vi "2636 EPSC fixed log time version.vi"() -> ()   [LabVIEW 2023]
uses:
  <instrlib>/Keithley 2600 Series/Public/Channel.ctl
  <instrlib>/Keithley 2600 Series/Keithley 2600 Series.lvlib
  <userlib>/_OpenG.lib/time/time.llb/openg_time.lvlib
panel:
  in  "Down Sample Factor":u8=3
  out "EPSC":cluster{"X":dbl[], "Y":dbl[]}[](graph)
  out "Log Time (s)":dbl=5000.0
  out "Gate Pulse":cluster{"X":dbl[], "Y":dbl[]}[](graph)
  in  "error in (no error)":errorcluster
  in  "Log Time Before Pulse (s)":dbl=0.5 format="%#_13g"
  in  "Log Time After Pulses (s)":dbl=10.0 format="%#_13g"
  in  "Auto Enable Output":bool=TRUE
  in  "Reset":bool=TRUE
  in  "Error Query":bool
  out "I_ds Points":i32=5000
  out "Pulsed IV Filename Out":path caption="Filename Out"
  in  "Pulsed IV Filename":path=path "C:/Data/pulse_I_V.lvm" caption="Filename"
  out "Pulse IV":cluster{"X":dbl[], "Y":dbl[]}[](graph)
  out "I_ds Log Filename Out":path caption="Filename Out"
  in  "I_ds Log Filename":path=path "C:/Data/I_ds_vs_time.lvm" caption="Filename"
  out "Data":dbl[](array[numeric])
  out "error out":errorcluster
  out "Complete?":bool
  out "Overrun?":bool
  out "Overflow?":bool
  in  "Stop":bool
  in  "Pulse Duration (s)":dbl=0.01
  in  "Post-Pulse Duration (s)":dbl=0.05
  in  "Pre-Pulse Duration (s)":dbl=0.05
  in  "Buffer size":u32=1024
  in  "Pulse Number":u32=10
  in  "Drain Source Channel":T1=enum."Channel B"
  in  "V_ds(V)":dbl=0.01
  in  "I_ds NPLC":dbl=0.1
  in  "I_ds Range (A)":dbl=1e-06
  in  "I pulse Range (A)":dbl=1e-06
  in  "I pulse NPLC":dbl=0.1
  in  "Pulse Level (V)":dbl=15.0
  in  "Pulse Channel":T1
  in  "2636 Address":refnum<visa-resource-name>="GPIB0::26::INSTR"
  # "Synaptic EPSC Measurement (Three-terminal Devices)"
  # "by JHC (20250308)"
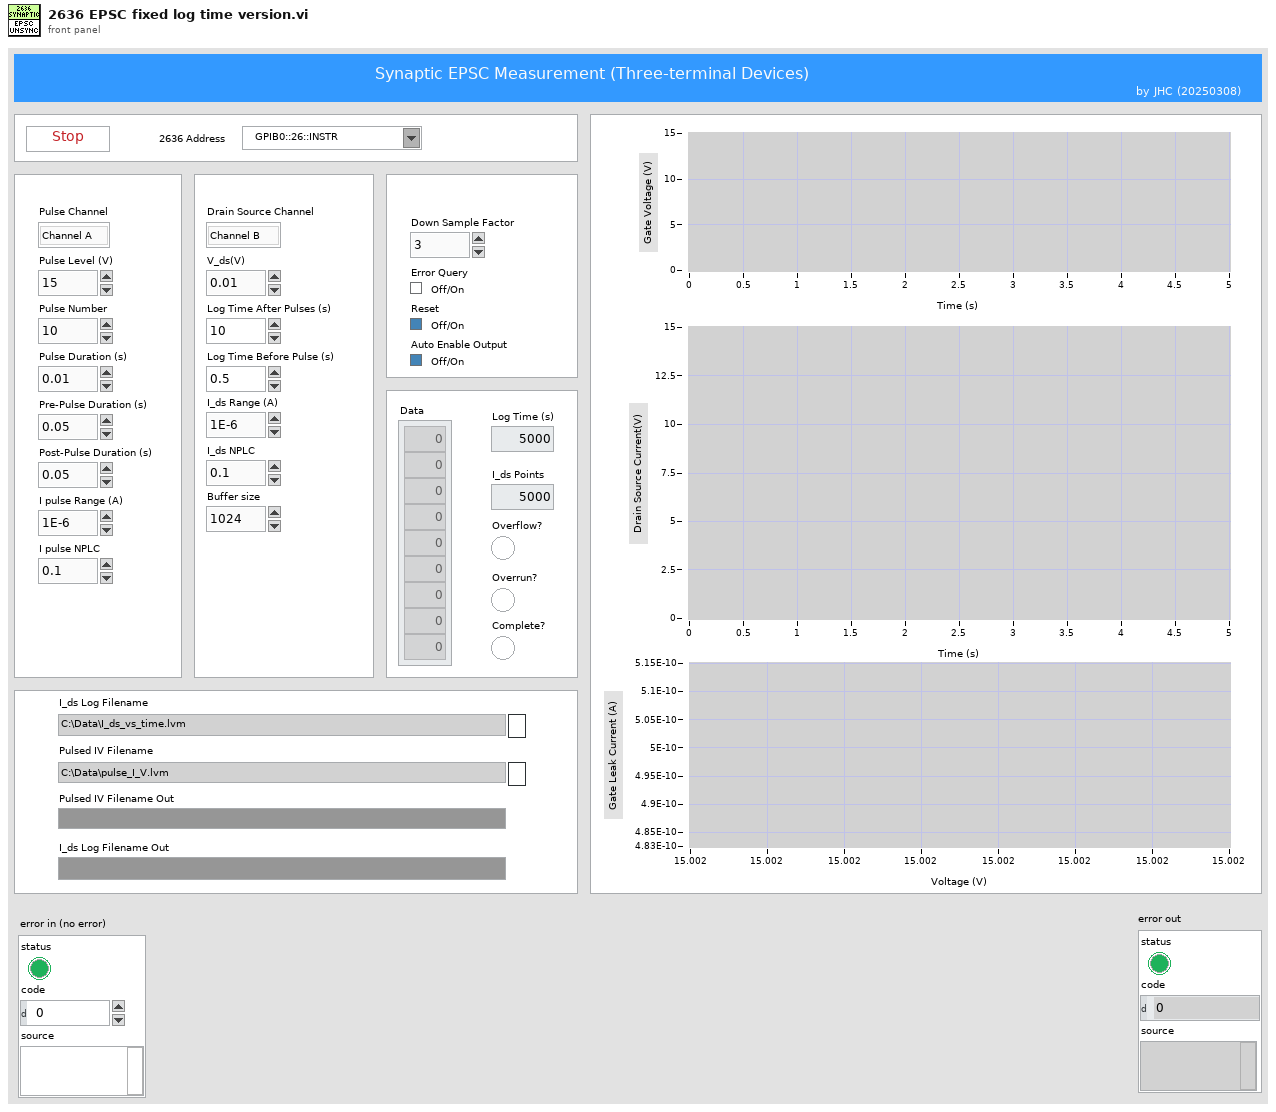
[diagram p1: front panel]
types:
  T1 = typedef "Keithley 2600 Series.lvlib/Channel.ctl" = enum32{"Channel A", "Channel B"}
  T2 = enum16{"None/Disconnect", "Digital I/O Trigger", "TSP-Link Trigger", "LAN Trigger", "Blender", "Timer Expired", "Front Panel Trigger", "Software Trigger", "SMU Sweeping", "SMU Armed", "SMU Source Complete", "SMU Measure Complete", "SMU Pulse Complete", "SMU Sweep Complete", "SMU Idle"}
  T3 = enum16{"Current", "Voltage", "IV", "Resistance", "Power"}
  T4 = enum32{"ASCII", "Real 32", "Real 64", "Single Precision Real", "Double Precision Real"}
  T5 = enum16{"Digital I/O", "TSP-Link", "LAN", "Blender", "Timer", "Arm", "Source", "Measure", "End Pulse"}
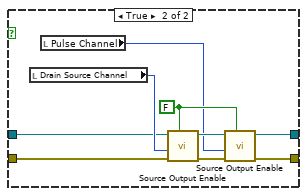
[diagram p2: hidden frame]
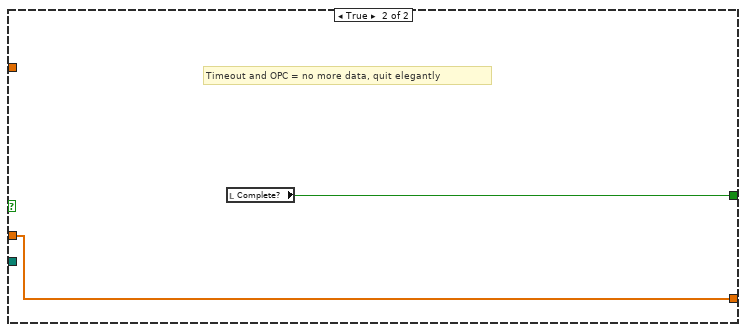
[diagram p5: hidden frame]
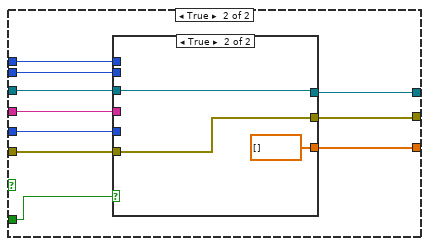
[diagram p8: hidden frame]
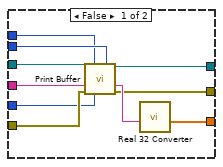
[diagram p9: hidden frame]
diagram:
  w25 = 0.0 ("element")
  w41 = sgl[] [] ("Data Array Out")
  w44 = u16 1 items=["Channel A", "Channel B"] ("Channel (Channel A)")
  w45 = u16 0 items=["Channel A", "Channel B"] ("Channel (Channel A)")
  w62 = u16 0 items=["Current", "Voltage", "Resistance", "Power"] ("Function (Current)")
  w70 = u16 2 items=["Channel A", "Channel B", "Channels A & B", "User"] ("Screen (Channels A & B)")
  # "Wait 1s"
  # "Start Pulse SMU"
  # "Start DS SMU"
  n1 = call <instrlib>:"Initialize.vi"("Reset (True)"="Reset", "error in (no error)"="error in (no error)", "Error Query (False)"="Error Query", "ID Query (True)"=TRUE, "VISA resource name"="2636 Address") -> ("error out"=w27:errorcluster, "VISA resource name out"=w30:refnum<visa-resource-name>)  [unwired: 5 in]
  n2 = call <instrlib>:"Error Queue Clear.vi"("error in (no error)"=w27, "VISA resource name"=w30) -> ("error out"=w28:errorcluster, "VISA resource name out"=w29:refnum<visa-resource-name>)  [unwired: 6 in, 2 out]
  n3 = call <instrlib>:"Abort SMU Op.vi"("error in"=w28, "Channel (Channel A)"=w45, "VISA resource name"=w29) -> ("error out"=w46:errorcluster, "VISA resource name out"=w47:refnum<visa-resource-name>)  [unwired: 5 in, 2 out]
  n4 = call <instrlib>:"Abort SMU Op.vi"("error in"=w46, "Channel (Channel A)"=w44, "VISA resource name"=w47) -> ("error out"=w42:errorcluster, "VISA resource name out"=w43:refnum<visa-resource-name>)  [unwired: 5 in, 2 out]
  n5 = call <instrlib>:"Reset SMU.vi"("SMU B (No)"="Reset", "SMU A (No)"="Reset", "error in (no error)"=w42, "VISA resource name"=w43) -> ("error out"=w109:errorcluster, "VISA resource name out"=w110:refnum<visa-resource-name>)  [unwired: 4 in, 2 out]
  n6 = flat-sequence {
    tunnel: w110 -> [w143]
    tunnel: w109 -> [w142]
    tunnel: [w124] -> w108
    tunnel: [w123] -> w107
    tunnel: w108 -> [w182]
    tunnel: w107 -> [w183]
    tunnel: [w181] -> w106
    tunnel: [w180] -> w105
    tunnel: w106 -> [w223]
    tunnel: w105 -> [w221]
    tunnel: [w202] -> w104
    tunnel: [w201] -> w103
    tunnel: w104 -> [w301]
    tunnel: w103 -> [w300]
    tunnel: [w268] -> w102
    tunnel: [w267] -> w101
    tunnel: [w253] -> w100
    tunnel: w102 -> [w326]
    tunnel: w101 -> [w327]
    tunnel: w100 -> [w352]
    tunnel: [w330] -> w99
    tunnel: [w329] -> w98
    tunnel: w99 -> [w360]
    tunnel: w98 -> [w359]
    tunnel: [w356] -> w67
    tunnel: [w355] -> w66
    frame #0 {
      w131 = enum32{"Current", "Voltage"}."Current" ("Function (Current)")
      w132 = FALSE ("Autorange (On)")
      w112 = enum32{"Current", "Voltage"}."Voltage" ("Function (Current)")
      # "Init Pulse Gate Channel"
      n7 = call <instrlib>:"Source Function.vi"("Function (Current)"=w112, "error in (no error)"=w142, "Channel (Channel A)"="Pulse Channel", "VISA resource name"=w143) -> ("error out"=w144:errorcluster, "VISA resource name out"=w145:refnum<visa-resource-name>)  [unwired: 4 in, 2 out]
      n8 = call <instrlib>:"Source Level.vi"("Level (0.000)"=0.0, "Function (Current)"=w112, "error in (no error)"=w144, "Channel (Channel A)"="Pulse Channel", "VISA resource name"=w145) -> ("error out"=w140:errorcluster, "VISA resource name out"=w141:refnum<visa-resource-name>)  [unwired: 3 in, 2 out]
      n9 = call <instrlib>:"Source Autorange.vi"("Autorange (On)"=w132, "Function (Current)"=w112, "error in (no error)"=w140, "Channel (Channel A)"="Pulse Channel", "VISA resource name"=w141) -> ("error out"=w138:errorcluster, "VISA resource name out"=w139:refnum<visa-resource-name>)  [unwired: 3 in, 2 out]
      n10 = local read "Pulse Level (V)"() -> (w111:dbl)
      n11 = call <instrlib>:"Source Autorange.vi"("Autorange (On)"=w132, "Function (Current)"=w131, "error in (no error)"=w138, "Channel (Channel A)"="Pulse Channel", "VISA resource name"=w139) -> ("error out"=w119:errorcluster, "VISA resource name out"=w121:refnum<visa-resource-name>)  [unwired: 3 in, 2 out]
      n12 = call <instrlib>:"Source Range.vi"("Range (1.000)"=w111, "Function (Current)"=w112, "error in (no error)"=w119, "Channel (Channel A)"="Pulse Channel", "VISA resource name"=w121) -> ("error out"=w118:errorcluster, "VISA resource name out"=w120:refnum<visa-resource-name>)  [unwired: 3 in, 2 out]
      n13 = call <instrlib>:"Measure NPLC.vi"("NPLC (1.000)"="I pulse NPLC", "error in (no error)"=w118, "Channel (Channel A)"="Pulse Channel", "VISA resource name"=w120) -> ("error out"=w136:errorcluster, "VISA resource name out"=w133:refnum<visa-resource-name>)  [unwired: 4 in, 2 out]
      n14 = call <instrlib>:"Measure Autorange.vi"("Autorange (On)"=w132, "Function (Current)"=w112, "error in (no error)"=w136, "Channel (Channel A)"="Pulse Channel", "VISA resource name"=w133) -> ("error out"=w135:errorcluster, "VISA resource name out"=w134:refnum<visa-resource-name>)  [unwired: 3 in, 2 out]
      n15 = call <instrlib>:"Measure Autorange.vi"("Autorange (On)"=w132, "Function (Current)"=w131, "error in (no error)"=w135, "Channel (Channel A)"="Pulse Channel", "VISA resource name"=w134) -> ("error out"=w117:errorcluster, "VISA resource name out"=w116:refnum<visa-resource-name>)  [unwired: 3 in, 2 out]
      n16 = call <instrlib>:"Measure Range.vi"("Range (1.000)"=w111, "Function (Current)"=w112, "error in (no error)"=w117, "Channel (Channel A)"="Pulse Channel", "VISA resource name"=w116) -> ("error out"=w114:errorcluster, "VISA resource name out"=w115:refnum<visa-resource-name>)  [unwired: 3 in, 2 out]
      n17 = call <instrlib>:"Measure Range.vi"("Range (1.000)"="I pulse Range (A)", "Function (Current)"=w131, "error in (no error)"=w114, "Channel (Channel A)"="Pulse Channel", "VISA resource name"=w115) -> ("error out"=w129:errorcluster, "VISA resource name out"=w128:refnum<visa-resource-name>)  [unwired: 3 in, 2 out]
      n18 = call <instrlib>:"Measure Sense Mode.vi"("error in (no error)"=w129, "Channel (Channel A)"="Pulse Channel", "VISA resource name"=w128) -> ("error out"=w126:errorcluster, "VISA resource name out"=w127:refnum<visa-resource-name>)  [unwired: 2 in, 5 out]
      n19 = call <instrlib>:"Measure Autozero.vi"("Autozero (Auto)"=enum32{"Off", "Once", "Auto"}."Once", "error in (no error)"=w126, "Channel (Channel A)"="Pulse Channel", "VISA resource name"=w127) -> ("error out"=w123:errorcluster, "VISA resource name out"=w124:refnum<visa-resource-name>)  [unwired: 1 in, 5 out]
    }
    frame #1 {
      w165 = 0.0 ("Interval (0.000)")
      w185 = enum32{"Current", "Voltage"}."Current" ("Function (Current)")
      w184 = FALSE ("Autorange (On)")
      w171 = enum32{"Current", "Voltage"}."Voltage" ("Function (Current)")
      # "50HZ"
      # "Init Drain Source Channel"
      n20 = local read "Log Time After Pulses (s)"() -> (w153:dbl)
      n21 = local read "Log Time Before Pulse (s)"() -> (w147:dbl)
      n22 = local read "Pulse Number"() -> (w152:u32)
      n23 = local read "Pre-Pulse Duration (s)"() -> (w148:dbl)
      n24 = local read "Pulse Duration (s)"() -> (w149:dbl)
      n25 = local read "Post-Pulse Duration (s)"() -> (w150:dbl)
      n26 = Compound Arithmetic op=ADD(w148, w149, w150) -> (w151:dbl)
      n27 = call <instrlib>:"Source Function.vi"("Function (Current)"=w171, "error in (no error)"=w183, "Channel (Channel A)"="Drain Source Channel", "VISA resource name"=w182) -> ("error out"=w199:errorcluster, "VISA resource name out"=w200:refnum<visa-resource-name>)  [unwired: 4 in, 2 out]
      n28 = Multiply(x=w152, y=w151) -> (x*y=w154:dbl)
      n29 = call <instrlib>:"Source Level.vi"("Level (0.000)"="V_ds(V)", "Function (Current)"=w171, "error in (no error)"=w199, "Channel (Channel A)"="Drain Source Channel", "VISA resource name"=w200) -> ("error out"=w197:errorcluster, "VISA resource name out"=w198:refnum<visa-resource-name>)  [unwired: 3 in, 2 out]
      n30 = Compound Arithmetic op=ADD(w153, w147, w154) -> (w146:dbl)
      "Log Time (s)" <- w146
      n31 = call <instrlib>:"Source Autorange.vi"("Autorange (On)"=w184, "Function (Current)"=w171, "error in (no error)"=w197, "Channel (Channel A)"="Drain Source Channel", "VISA resource name"=w198) -> ("error out"=w195:errorcluster, "VISA resource name out"=w196:refnum<visa-resource-name>)  [unwired: 3 in, 2 out]
      n32 = local read "I_ds NPLC"() -> (w159:dbl)
      n33 = call <instrlib>:"Source Autorange.vi"("Autorange (On)"=w184, "Function (Current)"=w185, "error in (no error)"=w195, "Channel (Channel A)"="Drain Source Channel", "VISA resource name"=w196) -> ("error out"=w179:errorcluster, "VISA resource name out"=w176:refnum<visa-resource-name>)  [unwired: 3 in, 2 out]
      n34 = Multiply(x=0.02, y=w159) -> (x*y=w157:dbl)
      n35 = call <instrlib>:"Source Range.vi"("Range (1.000)"="V_ds(V)", "Function (Current)"=w171, "error in (no error)"=w179, "Channel (Channel A)"="Drain Source Channel", "VISA resource name"=w176) -> ("error out"=w178:errorcluster, "VISA resource name out"=w177:refnum<visa-resource-name>)  [unwired: 3 in, 2 out]
      n36 = Divide(x=w146, y=w157) -> (x/y=w156:dbl)
      n37 = call <instrlib>:"Measure NPLC.vi"("NPLC (1.000)"="I_ds NPLC", "error in (no error)"=w178, "Channel (Channel A)"="Drain Source Channel", "VISA resource name"=w177) -> ("error out"=w166:errorcluster, "VISA resource name out"=w167:refnum<visa-resource-name>)  [unwired: 4 in, 2 out]
      n38 = To Long Integer(number=w156) -> (32bit integer=w155:i32)
      "I_ds Points" <- w155
      n39 = call <instrlib>:"Measure Interval.vi"("Interval (0.000)"=w165, "error in (no error)"=w166, "Channel (Channel A)"="Drain Source Channel", "VISA resource name"=w167) -> ("error out"=w169:errorcluster, "VISA resource name out"=w168:refnum<visa-resource-name>)  [unwired: 4 in, 2 out]
      n40 = call <instrlib>:"Measure Delay.vi"("Delay (0)"=w165, "error in (no error)"=w169, "Channel (Channel A)"="Drain Source Channel", "VISA resource name"=w168) -> ("error out"=w163:errorcluster, "VISA resource name out"=w164:refnum<visa-resource-name>)  [unwired: 4 in, 2 out]
      n41 = call <instrlib>:"Measure Count.vi"("Count (1)"=w155, "error in (no error)"=w163, "Channel (Channel A)"="Drain Source Channel", "VISA resource name"=w164) -> ("error out"=w161:errorcluster, "VISA resource name out"=w162:refnum<visa-resource-name>)  [unwired: 4 in, 2 out]
      n42 = call <instrlib>:"Measure Autorange.vi"("Autorange (On)"=w184, "Function (Current)"=w171, "error in (no error)"=w161, "Channel (Channel A)"="Drain Source Channel", "VISA resource name"=w162) -> ("error out"=w193:errorcluster, "VISA resource name out"=w192:refnum<visa-resource-name>)  [unwired: 3 in, 2 out]
      n43 = call <instrlib>:"Measure Autorange.vi"("Autorange (On)"=w184, "Function (Current)"=w185, "error in (no error)"=w193, "Channel (Channel A)"="Drain Source Channel", "VISA resource name"=w192) -> ("error out"=w172:errorcluster, "VISA resource name out"=w173:refnum<visa-resource-name>)  [unwired: 3 in, 2 out]
      n44 = call <instrlib>:"Measure Range.vi"("Range (1.000)"="V_ds(V)", "Function (Current)"=w171, "error in (no error)"=w172, "Channel (Channel A)"="Drain Source Channel", "VISA resource name"=w173) -> ("error out"=w175:errorcluster, "VISA resource name out"=w174:refnum<visa-resource-name>)  [unwired: 3 in, 2 out]
      n45 = call <instrlib>:"Measure Range.vi"("Range (1.000)"="I_ds Range (A)", "Function (Current)"=w185, "error in (no error)"=w175, "VISA resource name"=w174) -> ("error out"=w190:errorcluster, "VISA resource name out"=w189:refnum<visa-resource-name>)  [unwired: 4 in, 2 out]
      n46 = call <instrlib>:"Measure Sense Mode.vi"("error in (no error)"=w190, "Channel (Channel A)"="Drain Source Channel", "VISA resource name"=w189) -> ("error out"=w187:errorcluster, "VISA resource name out"=w188:refnum<visa-resource-name>)  [unwired: 2 in, 5 out]
      n47 = call <instrlib>:"Measure Autozero.vi"("Autozero (Auto)"=enum32{"Off", "Once", "Auto"}."Once", "error in (no error)"=w187, "Channel (Channel A)"="Drain Source Channel", "VISA resource name"=w188) -> ("error out"=w181:errorcluster, "VISA resource name out"=w180:refnum<visa-resource-name>)  [unwired: 1 in, 5 out]
    }
    frame #2 {
      w215 = TRUE ("Append Mode (Off)")
      w214 = "v_ds" ("Buffer Name (buf)")
      w216 = TRUE ("Append Mode (Off)")
      w218 = "i_ds" ("Buffer Name (buf)")
      w227 = FALSE ("Collect Timestamps (Off)")
      w226 = "pulse_iv_table.v" ("Buffer Name (buf)")
      w225 = TRUE ("Append Mode (Off)")
      w224 = "pulse_iv_table.i" ("Buffer Name (buf)")
      # "set up circular buffer"
      # "A large size"
      # "Init Buffer"
      n48 = local read "Pulse Channel"() -> (w242:T1)
      n49 = VISA Write(VISA resource name=w221, write buffer="pulse_iv_table = {}\nds_iv_table = {}", error in (no error)=w223) -> (VISA resource name out=w228:refnum<visa-resource-name>, error out=w229:errorcluster)  [unwired: 1 out]
      n50 = call <instrlib>:"Error Query.vi"("error in (no error)"=w229, "VISA resource name"=w228) -> ("error out"=w241:errorcluster, "VISA resource name out"=w240:refnum<visa-resource-name>)  [unwired: 8 out]
      n51 = call <instrlib>:"Buffer Make Buffer.vi"("Capacity (1)"="Pulse Number", "Channel (Channel A)"=w242, "error in (no error)"=w241, "Buffer Name (buf)"=w224, "VISA resource name"=w240) -> ("error out"=w230:errorcluster, "VISA resource name out"=w231:refnum<visa-resource-name>)  [unwired: 1 in, 4 out]
      n52 = call <instrlib>:"Buffer Clear.vi"("error in (no error)"=w230, "Buffer Name"=w224, "VISA resource name"=w231) -> ("error out"=w233:errorcluster, "VISA resource name out"=w232:refnum<visa-resource-name>)  [unwired: 7 out]
      n53 = call <instrlib>:"Buffer Configure.vi"("Collect Timestamps (Off)"=w227, "error in (no error)"=w233, "Buffer Name"=w224, "Append Mode (Off)"=w225, "VISA resource name"=w232) -> ("error out"=w235:errorcluster, "VISA resource name out"=w234:refnum<visa-resource-name>)  [unwired: 2 in, 3 out]
      n54 = call <instrlib>:"Buffer Make Buffer.vi"("Capacity (1)"="Pulse Number", "Channel (Channel A)"=w242, "error in (no error)"=w235, "Buffer Name (buf)"=w226, "VISA resource name"=w234) -> ("error out"=w237:errorcluster, "VISA resource name out"=w236:refnum<visa-resource-name>)  [unwired: 1 in, 4 out]
      n55 = call <instrlib>:"Buffer Clear.vi"("error in (no error)"=w237, "Buffer Name"=w226, "VISA resource name"=w236) -> ("error out"=w239:errorcluster, "VISA resource name out"=w238:refnum<visa-resource-name>)  [unwired: 7 out]
      n56 = call <instrlib>:"Buffer Configure.vi"("Collect Source Values (Off)"=w227, "error in (no error)"=w239, "Buffer Name"=w226, "Append Mode (Off)"=w225, "VISA resource name"=w238) -> ("error out"=w249:errorcluster, "VISA resource name out"=w248:refnum<visa-resource-name>)  [unwired: 2 in, 3 out]
      n57 = local read "Drain Source Channel"() -> (w206:T1)
      n58 = call <instrlib>:"Buffer Make Buffer.vi"("Capacity (1)"="Buffer size", "Channel (Channel A)"=w206, "error in (no error)"=w249, "Buffer Name (buf)"=w218, "VISA resource name"=w248) -> ("error out"=w245:errorcluster, "VISA resource name out"=w244:refnum<visa-resource-name>)  [unwired: 1 in, 4 out]
      n59 = call <instrlib>:"Buffer Clear.vi"("error in (no error)"=w245, "Buffer Name"=w218, "VISA resource name"=w244) -> ("error out"=w247:errorcluster, "VISA resource name out"=w246:refnum<visa-resource-name>)  [unwired: 7 out]
      n60 = call <instrlib>:"Buffer Configure.vi"("Collect Timestamps (Off)"=w216, "error in (no error)"=w247, "Buffer Name"=w218, "Append Mode (Off)"=w216, "VISA resource name"=w246) -> ("error out"=w220:errorcluster, "VISA resource name out"=w219:refnum<visa-resource-name>)  [unwired: 2 in, 3 out]
      n61 = call <instrlib>:"Advanced Buffer Configuration.vi"("VISA resource name"=w219, "Enable Buffer Cache Mode (Disable)"=w216, "Buffer Name"=w218, "Buffer Fill Mode (Fill_Once)"=enum16{"FILL_ONCE", "FILL_WINDOW"}."FILL_WINDOW", "error in (no error)"=w220) -> ("VISA resource name out"=w204:refnum<visa-resource-name>, "error out"=w203:errorcluster)  [unwired: 9 in]
      n62 = call <instrlib>:"Buffer Make Buffer.vi"("Capacity (1)"="Buffer size", "Channel (Channel A)"=w206, "error in (no error)"=w203, "Buffer Name (buf)"=w214, "VISA resource name"=w204) -> ("error out"=w210:errorcluster, "VISA resource name out"=w211:refnum<visa-resource-name>)  [unwired: 1 in, 4 out]
      n63 = call <instrlib>:"Buffer Clear.vi"("error in (no error)"=w210, "Buffer Name"=w214, "VISA resource name"=w211) -> ("error out"=w208:errorcluster, "VISA resource name out"=w209:refnum<visa-resource-name>)  [unwired: 7 out]
      n64 = call <instrlib>:"Buffer Configure.vi"("Collect Timestamps (Off)"=w215, "error in (no error)"=w208, "Buffer Name"=w214, "Append Mode (Off)"=w215, "VISA resource name"=w209) -> ("error out"=w212:errorcluster, "VISA resource name out"=w213:refnum<visa-resource-name>)  [unwired: 2 in, 3 out]
      n65 = call <instrlib>:"Advanced Buffer Configuration.vi"("VISA resource name"=w213, "Enable Buffer Cache Mode (Disable)"=w215, "Buffer Name"=w214, "Buffer Fill Mode (Fill_Once)"=enum16{"FILL_ONCE", "FILL_WINDOW"}."FILL_WINDOW", "error in (no error)"=w212) -> ("VISA resource name out"=w201:refnum<visa-resource-name>, "error out"=w202:errorcluster)  [unwired: 9 in]
    }
    frame #3 {
      w257 = u32 4 ("Timer Number (1)")
      w271 = u32 1 ("Timer Number (1)")
      w283 = u32 3 ("Timer Number (1)")
      w307 = u32 2 ("Timer Number (1)")
      # "SMU Armed when timer4 expires"
      # "Trigger timer4 when the SMU Sweeping, only once"
      # "Trigger timer1 when the SMU Armed, repeat N times"
      # "Trigger end pulse after timer3 expired"
      # "Configure measure action (default is 0) to start after source immediately"
      # "set source pulse level and end pusle idle"
      # "Trigger timer3 when the SMU source pulse level"
      # "Create a fixed level voltage sweep"
      # "Configure source action to start after timer2 expired"
      # "Trigger timer2 when timer1 expired or first run."
      # "Init Trigger Model (Pulse Channel)"
      n66 = local read "Pulse Channel"() -> (w253:T1)
      n67 = Pick Line(multi-line string="smua\nsmub", line index=w253) -> (output string=w266:string)  [unwired: 1 in]
      n68 = Format Into String(format string="%s.trigger.source.listv({%f})\\n", w266, "Pulse Level (V)") -> (resulting string=w304:string)  [unwired: 2 in, 1 out]
      n69 = call <instrlib>:"Format Event ID.vi"("Channel (Channel A)"=w253, "Event Type (None)"=T2."SMU Sweeping") -> ("Event ID"=w261:string)  [unwired: 8 in, 1 out]
      n70 = Format Into String(format string="%s.trigger.source.action = %s.ENABLE\n%s.trigger.endpulse.action = %s.SOURCE_IDLE", initial string=w304, w266, w266, w266, w266) -> (resulting string=w299:string)  [unwired: 1 in, 1 out]
      n71 = VISA Write(VISA resource name=w300, write buffer=w299, error in (no error)=w301) -> (VISA resource name out=w263:refnum<visa-resource-name>, error out=w262:errorcluster)  [unwired: 1 out]
      n72 = call <instrlib>:"Config Timer.vi"("VISA resource name"=w263, "Delay (1e-3)"="Log Time Before Pulse (s)", "Timer Number (1)"=w257, "error in"=w262, "Input Event"=w261) -> ("VISA resource name out"=w259:refnum<visa-resource-name>, "error out"=w255:errorcluster)  [unwired: 7 in, 2 out]
      n73 = call <instrlib>:"Format Event ID.vi"("Event Module # (1)"=w257, "Event Type (None)"=T2."Timer Expired") -> ("Event ID"=w256:string)  [unwired: 8 in, 1 out]
      n74 = call <instrlib>:"Config Arm Event.vi"("Arm Input Event"=w256, "error in"=w255, "Channel (Channel A)"=w253, "VISA resource name"=w259) -> ("error out"=w251:errorcluster, "VISA resource name out"=w250:refnum<visa-resource-name>)  [unwired: 4 in, 2 out]
      n75 = call <instrlib>:"Format Event ID.vi"("Channel (Channel A)"=w253, "Event Type (None)"=T2."SMU Armed") -> ("Event ID"=w252:string)  [unwired: 8 in, 1 out]
      n76 = local read "Pre-Pulse Duration (s)"() -> (w280:dbl)
      n77 = local read "Pulse Number"() -> (w276:u32)
      n78 = local read "Pulse Duration (s)"() -> (w281:dbl)
      n79 = Decrement(x=w276) -> (x-1=w272:u32)
      n80 = Compound Arithmetic op=ADD(w281, w280, "Post-Pulse Duration (s)") -> (w278:dbl)
      n81 = call <instrlib>:"Config Timer.vi"("VISA resource name"=w250, "Count (1)"=w272, "Delay (1e-3)"=w278, "Timer Number (1)"=w271, "Passthrough (Off)"=TRUE, "error in"=w251, "Input Event"=w252) -> ("VISA resource name out"=w273:refnum<visa-resource-name>, "error out"=w274:errorcluster)  [unwired: 5 in, 2 out]
      n82 = call <instrlib>:"Format Event ID.vi"("Event Module # (1)"=w271, "Event Type (None)"=T2."Timer Expired") -> ("Event ID"=w311:string)  [unwired: 8 in, 1 out]
      n83 = call <instrlib>:"Config Timer.vi"("VISA resource name"=w273, "Delay (1e-3)"="Pre-Pulse Duration (s)", "Timer Number (1)"=w307, "error in"=w274, "Input Event"=w311) -> ("VISA resource name out"=w310:refnum<visa-resource-name>, "error out"=w309:errorcluster)  [unwired: 7 in, 2 out]
      n84 = call <instrlib>:"Format Event ID.vi"("Event Module # (1)"=w307, "Event Type (None)"=T2."Timer Expired") -> ("Event ID"=w306:string)  [unwired: 8 in, 1 out]
      n85 = call <instrlib>:"Config Source Event.vi"("Input Event"=w306, "error in"=w309, "Channel (Channel A)"=w253, "VISA resource name"=w310) -> ("error out"=w294:errorcluster, "VISA resource name out"=w295:refnum<visa-resource-name>)  [unwired: 4 in, 2 out]
      n86 = call <instrlib>:"Format Event ID.vi"("Channel (Channel A)"=w253, "Event Type (None)"=T2."SMU Source Complete") -> ("Event ID"=w297:string)  [unwired: 8 in, 1 out]
      n87 = call <instrlib>:"Config Timer.vi"("VISA resource name"=w295, "Delay (1e-3)"="Pulse Duration (s)", "Timer Number (1)"=w283, "error in"=w294, "Input Event"=w297) -> ("VISA resource name out"=w293:refnum<visa-resource-name>, "error out"=w292:errorcluster)  [unwired: 7 in, 2 out]
      n88 = call <instrlib>:"Config Measure Event.vi"("VISA resource name"=w293, "Configure Measurement (Disable)"=enum8{"DISABLE", "ENABLE", "ASYNC"}."ENABLE", "Buffer 1"="pulse_iv_table.i" ("Buffer Name (buf)"), "Buffer 2"="pulse_iv_table.v" ("Buffer Name (buf)"), "Channel (Channel A)"=w253, "Function (Current)"=T3."IV", "error in"=w292, "Measure Input Event"="0") -> ("VISA resource name out"=w286:refnum<visa-resource-name>, "error out"=w285:errorcluster)  [unwired: 4 in, 2 out]
      n89 = call <instrlib>:"Format Event ID.vi"("Event Module # (1)"=w283, "Event Type (None)"=T2."Timer Expired") -> ("Event ID"=w282:string)  [unwired: 8 in, 1 out]
      n90 = local read "Pulse Number"() -> (w264:u32)
      n91 = call <instrlib>:"Config End Pulse Event.vi"("Input Event"=w282, "error in"=w285, "Channel (Channel A)"=w253, "VISA resource name"=w286) -> ("error out"=w270:errorcluster, "VISA resource name out"=w269:refnum<visa-resource-name>)  [unwired: 4 in, 2 out]
      n92 = call <instrlib>:"Config Layer Count.vi"("Trigger Count (1)"=w264, "Arm Count (1)"=u32 1 ("Trigger Count (1)"), "error in"=w270, "Channel (Channel A)"=w253, "VISA resource name"=w269) -> ("error out"=w267:errorcluster, "VISA resource name out"=w268:refnum<visa-resource-name>)  [unwired: 3 in, 2 out]
    }
    frame #4 {
      w331 = u32 1 ("Arm Count (1)")
      w340 = u32 1 ("Blender Number (1)")
      # "BUG from Driver: if Async, measure.Y is not set"
      # "timer4 to trigger async measure action"
      # "Trigger timer4 when SMU source complete,\npassthrough so measure right after that"
      # "Blend two events from Pulse SMU trigger DS SMU Source action\nDS SMU Source start when Pulse SMU start sweeping\nWhen Pulse SMU become idle, DS SMU source again and stop"
      # "set source level, and hold"
      # "Create a fixed level voltage sweep"
      # "Init Trigger Model (Drain Source Channel)"
      n93 = local read "Drain Source Channel"() -> (w332:T1)
      n94 = local read "V_ds(V)"() -> (w344:dbl)
      n95 = Pick Line(multi-line string="smua\nsmub", line index=w332) -> (output string=w317:string)  [unwired: 1 in]
      n96 = Format Into String(format string="%s.trigger.source.listv({%f})\\n", w317, w344) -> (resulting string=w347:string)  [unwired: 2 in, 1 out]
      n97 = call <instrlib>:"Format Event ID.vi"("Channel (Channel A)"=w352, "Event Type (None)"=T2."SMU Sweeping") -> ("Event ID"=w350:string)  [unwired: 8 in, 1 out]
      n98 = Format Into String(format string="%s.trigger.source.action = %s.ENABLE\n%s.trigger.endpulse.action = %s.SOURCE_HOLD", initial string=w347, w317, w317, w317, w317) -> (resulting string=w323:string)  [unwired: 1 in, 1 out]
      n99 = call <instrlib>:"Format Event ID.vi"("Channel (Channel A)"=w352, "Event Type (None)"=T2."SMU Sweep Complete") -> ("Event ID"=w349:string)  [unwired: 8 in, 1 out]
      n100 = VISA Write(VISA resource name=w326, write buffer=w323, error in (no error)=w327) -> (VISA resource name out=w325:refnum<visa-resource-name>, error out=w324:errorcluster)  [unwired: 1 out]
      n101 = call <instrlib>:"Config Event Blender.vi"("VISA resource name"=w325, "Input Event 1"=w350, "Input Event 2"=w349, "Blender Number (1)"=w340, "Blend Type (OR)"=enum16{"OR", "AND"}."OR", "error in"=w324) -> ("VISA resource name out"=w342:refnum<visa-resource-name>, "error out"=w343:errorcluster)  [unwired: 6 in, 2 out]
      n102 = call <instrlib>:"Format Event ID.vi"("Event Module # (1)"=w340, "Event Type (None)"=T2."Blender") -> ("Event ID"=w339:string)  [unwired: 8 in, 1 out]
      n103 = call <instrlib>:"Config Source Event.vi"("Input Event"=w339, "error in"=w343, "Channel (Channel A)"=w332, "VISA resource name"=w342) -> ("error out"=w335:errorcluster, "VISA resource name out"=w336:refnum<visa-resource-name>)  [unwired: 4 in, 2 out]
      n104 = call <instrlib>:"Format Event ID.vi"("Channel (Channel A)"=w332, "Event Type (None)"=T2."SMU Armed") -> ("Event ID"=w315:string)  [unwired: 8 in, 1 out]
      n105 = call <instrlib>:"Config Measure Event.vi"("VISA resource name"=w336, "Configure Measurement (Disable)"=enum8{"DISABLE", "ENABLE", "ASYNC"}."ENABLE", "Buffer 1"="i_ds" ("Buffer Name (buf)"), "Buffer 2"="v_ds" ("Buffer Name (buf)"), "Channel (Channel A)"=w332, "Function (Current)"=T3."IV", "error in"=w335, "Measure Input Event"=w315) -> ("VISA resource name out"=w319:refnum<visa-resource-name>, "error out"=w320:errorcluster)  [unwired: 4 in, 2 out]
      n106 = Format Into String(format string="%s.trigger.measure.action = %s.ASYNC", w317, w317) -> (resulting string=w316:string)  [unwired: 2 in, 1 out]
      n107 = VISA Write(VISA resource name=w319, write buffer=w316, error in (no error)=w320) -> (VISA resource name out=w322:refnum<visa-resource-name>, error out=w321:errorcluster)  [unwired: 1 out]
      n108 = call <instrlib>:"Config Layer Count.vi"("Trigger Count (1)"=w331, "Arm Count (1)"=w331, "error in"=w321, "Channel (Channel A)"=w332, "VISA resource name"=w322) -> ("error out"=w329:errorcluster, "VISA resource name out"=w330:refnum<visa-resource-name>)  [unwired: 3 in, 2 out]
    }
    frame #5 {
      # "Other init jobs"
      n109 = call <instrlib>:"Data Output Format.vi"("ASCII Precision (6)"=6, "error in (no error)"=w359, "Data Format (ASCII)"=T4."Real 32", "VISA resource name"=w360) -> ("error out"=w355:errorcluster, "VISA resource name out"=w356:refnum<visa-resource-name>)  [unwired: 4 in, 2 out]
    }
  }
  n110 = local read "Log Time Before Pulse (s)"() -> (w21:dbl)
  n111 = local read "Post-Pulse Duration (s)"() -> (w17:dbl)
  n112 = local read "Pre-Pulse Duration (s)"() -> (w20:dbl)
  n113 = local read "Log Time After Pulses (s)"() -> (w7:dbl)
  n114 = local read "Pulse Duration (s)"() -> (w18:dbl)
  n115 = local read "Pulse Level (V)"() -> (w19:dbl)
  n116 = local read "Pulse Channel"() -> (w64:T1)
  n117 = local read "Drain Source Channel"() -> (w63:T1)
  n118 = Build Array(w25, w21) -> (w23:dbl[])
  n119 = local read "Pulse Number"() -> (w24:u32)
  n120 = Build Array(w25, w25) -> (w22:dbl[])
  n121 = call <instrlib>:"Display Screen.vi"("Screen (Channels A & B)"=w70, "error in (no error)"=w66, "VISA resource name"=w67) -> ("error out"=w73:errorcluster, "Node Out"=w72:string, "VISA resource name out"=w71:refnum<visa-resource-name>)  [unwired: 5 in, 1 out]
  n122 = for {
    N: w24 -> [_]
    shift-right: [w369] -> w16
    shift-left: w22 -> [w370]
    shift-right: [w371] -> w15
    shift-left: w23 -> [w372]
    tunnel: w20 -> [w366]
    tunnel: w19 -> [w361]
    tunnel: w18 -> [w368]
    shift-right: [w363] -> w8
    shift-left: w21 -> [w373]
    tunnel: w17 -> [w367]
    w365 = 0.0 ("element")
    n123 = Add(x=w373, y=w366) -> (x+y=w364:dbl)
    n124 = Add(x=w364, y=w368) -> (x+y=w362:dbl)
    n125 = Add(x=w362, y=w367) -> (x+y=w363:dbl)
    n126 = Build Array (concatenate)(w370, w365, w361, w361, w365, w365) -> (w369:dbl[])
    n127 = Build Array (concatenate)(w372, w364, w364, w362, w362, w363) -> (w371:dbl[])
  }
  n128 = call <instrlib>:"Display Measure Function.vi"("Function (Current)"=w62, "error in (no error)"=w73, "Channel (Channel A)"=w64, "Node In"=w72, "VISA resource name"=w71) -> ("error out"=w69:errorcluster, "VISA resource name out"=w68:refnum<visa-resource-name>)  [unwired: 3 in, 2 out]
  n129 = control-ref of="Overflow?"() -> (w59:refnum<vi>)
  n130 = control-ref of="Overrun?"() -> (w58:refnum<vi>)
  n131 = control-ref of="Complete?"() -> (w57:refnum<vi>)
  n132 = control-ref of="Stop"() -> (w52:refnum<vi>)
  n133 = call <instrlib>:"Display Measure Function.vi"("Function (Current)"=w62, "error in (no error)"=w69, "Channel (Channel A)"=w63, "VISA resource name"=w68) -> ("error out"=w65:errorcluster, "VISA resource name out"=w61:refnum<visa-resource-name>)  [unwired: 4 in, 2 out]
  n134 = case shown="True" "Auto Enable Output" {
    tunnel: [w374 w384] -> w34
    tunnel: [w375 w383] -> w35
    tunnel: w65 -> [w374 w379]
    tunnel: w64 -> [_ w378]
    tunnel: w63 -> [_ w377]
    tunnel: w61 -> [w375 w376]
    frame False {
    }
    frame True {
      w380 = TRUE ("Output (Off)")
      n135 = call <instrlib>:"Source Output Enable.vi"("Output (Off)"=w380, "error in (no error)"=w379, "Channel (Channel A)"=w377, "VISA resource name"=w376) -> ("error out"=w382:errorcluster, "VISA resource name out"=w381:refnum<visa-resource-name>)  [unwired: 4 in, 2 out]
      n136 = call <instrlib>:"Source Output Enable.vi"("Output (Off)"=w380, "error in (no error)"=w382, "Channel (Channel A)"=w378, "VISA resource name"=w381) -> ("error out"=w384:errorcluster, "VISA resource name out"=w383:refnum<visa-resource-name>)  [unwired: 4 in, 2 out]
    }
  }
  n137 = Build Array(w59, w58, w57, w52) -> (w56:refnum<vi>[])
  n138 = for {
    tunnel: w56 -> [w386] mode=indexing
    tunnel: [w385] -> w53
    # "Init GUI"
    n139 = invoke class="Bool (strict)" method="Reinit To Default"(reference=w386) -> (error out=w385:errorcluster)  [unwired: 2 in, 2 out]
  }
  n140 = Add(x=w8, y=w7) -> (x+y=w6:dbl)
  n141 = Build Array (concatenate)(w16, 0.0 ("element")) -> (w13:dbl[])
  n142 = Build Array (concatenate)(w15, w6) -> (w12:dbl[])
  n143 = call "Convert to Dynamic Data5"("Array"=w12) -> ("Dynamic Data Type"=w10:dynamicdata)  [unwired: 3 in]
  n144 = call "Convert to Dynamic Data4"("Array"=w13) -> ("Dynamic Data Type"=w9:dynamicdata)  [unwired: 3 in]
  n145 = call <userlib>:"Wait (ms)__ogtk.vi"("error in (no error)"=w34, "milliseconds to wait"=u32 1000) -> ("error out"=w33:errorcluster)  [unwired: 8 in, 1 out]
  n146 = call "Build XY Graph2"("Y Input"=w9, "X Input"=w10) -> ("XY Graph"=→"Gate Pulse":cluster{"X":dbl[], "Y":dbl[]}[])  [unwired: 8 in, 1 out]
  n147 = call <instrlib>:"Initiate Sweep.vi"("error in"=w33, "Channel (Channel A)"=w63, "VISA resource name"=w35) -> ("error out"=w93:errorcluster, "VISA resource name out"=w94:refnum<visa-resource-name>)  [unwired: 5 in, 2 out]
  n148 = Obtain Queue(max queue size (-1, unlimited)=1024, name (unnamed)="data_q", element data type=w41, error in (no error)=w65) -> (queue out=w80:refnum<queue>, error out=w54:errorcluster)  [unwired: 1 in, 1 out]
  n149 = Format Into String(format string="%s, %s, %s", "i_ds" ("Buffer Name(s)"), "i_ds.timestamps" ("Buffer Name(s)"), "v_ds" ("Buffer Name(s)")) -> (resulting string=w97:string)  [unwired: 2 in, 1 out]
  n150 = call <instrlib>:"Initiate Sweep.vi"("error in"=w93, "Channel (Channel A)"=w64, "VISA resource name"=w94) -> ("error out"=w96:errorcluster, "VISA resource name out"=w95:refnum<visa-resource-name>)  [unwired: 5 in, 2 out]
  n151 = Merge Errors(w54, w53) -> (w55:errorcluster)
  n152 = while {
    tunnel: w80 -> [w398]
    tunnel: "I_ds Log Filename" -> [w394]
    tunnel: w55 -> [w397]
    tunnel: [w393] -> w51
    shift-right: [w387] -> w40
    shift-left: w41 -> [w388]
    stop <- w391 stop-if-true
    # "Plot and save I_ds and v_ds"
    n153 = Dequeue Element(queue=w398, timeout in ms (-1)=500, error in (no error)=w397) -> (queue out=w393:refnum<queue>, element=w395:sgl[], timed out?=w396:bool, error out=w390:errorcluster)
    n154 = case shown="False" w396 {
      tunnel: w395 -> [w410 _]
      tunnel: w394 -> [w416 _]
      tunnel: [FALSE ("Operation Complete") w427] -> w389
      tunnel: w388 -> [w411 w426]
      tunnel: [w409 w426] -> w387
      frame False {
        n155 = Decimate 1D Array(w410) -> (w406:sgl[], w407:sgl[], w414:sgl[])
        n156 = Build Array (concatenate)(w411, w410) -> (w409:sgl[])
        n157 = for {
          tunnel: [w424] -> w413 mode=indexing
          tunnel: w406 -> [w422] mode=indexing
          tunnel: w407 -> [w423] mode=indexing
          tunnel: w414 -> [w425] mode=indexing
          tunnel: [w424] -> w408
          tunnel: [w423] -> w401 mode=indexing if=w418
          tunnel: [w422] -> w400 mode=indexing if=w418
          tunnel: "Down Sample Factor" -> [w420]
          i -> [w421]
          n158 = Build Array(w423, w422, w425) -> (w424:sgl[])
          n159 = Quotient & Remainder(x=w421, y=w420) -> (x-y*floor(x/y)=w419:i32)  [unwired: 1 out]
          n160 = Equal To 0?(x=w419) -> (x = 0?=w418:bool)
        }
        "Data" <- w408
        n161 = call "Convert to Dynamic Data3"("2D Array"=w413) -> ("Dynamic Data Type"=w415:dynamicdata)  [unwired: 3 in]
        n162 = call "Write To Measurement File"("Signals"=w415, "Filename"=w416) -> ("Filename Out"=→"I_ds Log Filename Out":path)  [unwired: 15 in, 2 out]
        n163 = call "Convert to Dynamic Data6"("Array"=w401) -> ("Dynamic Data Type"=w404:dynamicdata)  [unwired: 3 in]
        n164 = call "Convert to Dynamic Data7"("Array"=w400) -> ("Dynamic Data Type"=w405:dynamicdata)  [unwired: 3 in]
        n165 = call "Build XY Graph3"("Y Input"=w405, "X Input"=w404) -> ("XY Graph"=→"EPSC":cluster{"X":dbl[], "Y":dbl[]}[])  [unwired: 8 in, 1 out]
      }
      frame True {
        # "Timeout and OPC = no more data, quit elegantly"
        n166 = local read "Complete?"() -> (w427:bool)
      }
    }
    n167 = local read "Stop"() -> (w392:bool)
    n168 = Compound Arithmetic op=OR(w389, w392, w390) -> (w391:bool)
  }
  n169 = while {
    tunnel: w95 -> [w437]
    tunnel: w96 -> [w436]
    shift-right: [w430] -> _
    shift-left: u32 1 ("Start Index (1)") -> [w429]
    tunnel: w97 -> [w457]
    tunnel: "tostring(i_ds.next), tostring(v_ds.next)" ("format string") -> [w455]
    tunnel: w80 -> [w435]
    tunnel: [w439] -> w84
    tunnel: [w433] -> w83
    tunnel: [w438] -> w76
    stop <- w440 stop-if-true
    # "Fetch buffer data and parse dataframes"
    n170 = Wait (ms)(milliseconds to wait=u32 100) -> ()  [unwired: 1 out]
    n171 = VISA Write(VISA resource name=w437, write buffer="*OPC", error in (no error)=w436) -> (VISA resource name out=w450:refnum<visa-resource-name>, error out=w449:errorcluster)  [unwired: 1 out]
    n172 = call <instrlib>:"ESR.vi"("error in (no error)"=w449, "VISA resource name"=w450) -> ("error out"=w444:errorcluster, "ESR"=w448:u8, "VISA resource name out"=w443:refnum<visa-resource-name>)  [unwired: 5 in, 2 out]
    n173 = And(x=w448, y=u8 1) -> (x .and. y?=w447:u8)
    n174 = Not Equal To 0?(x=w447) -> (x != 0?=w438:bool)
    "Complete?" <- w438
    n175 = call <instrlib>:"Print.vi"("Byte Count (1024)"=u32 256, "error in (no error)"=w444, "Input"=w455, "VISA resource name"=w443) -> ("error out"=w464:errorcluster, "Output"=w466:string, "VISA resource name out"=w461:refnum<visa-resource-name>)  [unwired: 3 in, 2 out]
    n176 = Scan From String(format string="%d %d", input string=w466, error in=w464) -> (error out=w460:errorcluster, output 1=w463:i32, output 2=w462:i32)  [unwired: 3 in, 2 out]
    n177 = Max & Min(x=w463, y=w462) -> (min(x,y)=w430:i32)  [unwired: 1 out]
    n178 = Decrement(x=w430) -> (x-1=w442:i32)
    n179 = Greater Or Equal?(x=w430, y=w429) -> (x >= y?=w459:bool)
    n180 = Equal?(x=w430, y=w429) -> (x = y?=w428:bool)
    n181 = case shown="False" w459 {
      tunnel: w457 -> [w473 w500]
      tunnel: w461 -> [w476 w499]
      tunnel: w460 -> [w477 w498]
      tunnel: w442 -> [w483 w497]
      tunnel: w429 -> [w490 w496]
      tunnel: u32 4096 ("Byte Count (1024)") -> [w489 w495]
      tunnel: [w479 w494] -> w432
      tunnel: [w472 w492] -> w434
      tunnel: [w471 w493] -> w454
      tunnel: w428 -> [_ w491]
      frame False {
        n182 = VISA Write(VISA resource name=w476, write buffer="i_ds.clearcache()\nv_ds.clearcache()" ("format string"), error in (no error)=w477) -> (VISA resource name out=w475:refnum<visa-resource-name>, error out=w474:errorcluster)  [unwired: 1 out]
        n183 = local read "Buffer size"() -> (w488:u32)
        n184 = call <instrlib>:"Print Buffer.vi"("VISA resource name"=w475, "Start Index (1)"=w490, "End Index (1)"=w488, "Buffer Name(s)"=w473, "error in (no error)"=w474, "Byte Count (1024)"=w489) -> ("VISA resource name out"=w486:refnum<visa-resource-name>, "Buffer Data"=w487:string, "error out"=w485:errorcluster)  [unwired: 5 in, 2 out]
        n185 = call <instrlib>:"Real 32 Converter.vi"("Data In"=w487) -> ("Data Array Out"=w481:sgl[])  [unwired: 10 in]
        n186 = call <instrlib>:"Print Buffer.vi"("VISA resource name"=w486, "Start Index (1)"=u32 1, "End Index (1)"=w483, "Buffer Name(s)"=w473, "error in (no error)"=w485) -> ("VISA resource name out"=w471:refnum<visa-resource-name>, "Buffer Data"=w482:string, "error out"=w472:errorcluster)  [unwired: 6 in, 2 out]
        n187 = call <instrlib>:"Real 32 Converter.vi"("Data In"=w482) -> ("Data Array Out"=w480:sgl[])  [unwired: 10 in]
        n188 = Build Array (concatenate)(w481, w480) -> (w479:sgl[])
      }
      frame True {
        n189 = case shown="True" w491 {
          tunnel: w500 -> [w510 _]
          tunnel: w499 -> [w509 w513]
          tunnel: w498 -> [w508 w512]
          tunnel: w497 -> [w507 _]
          tunnel: w496 -> [w506 _]
          tunnel: w495 -> [w505 _]
          tunnel: [w503 sgl[] [] ("Data Array Out")] -> w494
          tunnel: [w502 w513] -> w493
          tunnel: [w501 w512] -> w492
          frame False {
            n190 = call <instrlib>:"Print Buffer.vi"("VISA resource name"=w509, "Start Index (1)"=w506, "End Index (1)"=w507, "Buffer Name(s)"=w510, "error in (no error)"=w508, "Byte Count (1024)"=w505) -> ("VISA resource name out"=w502:refnum<visa-resource-name>, "Buffer Data"=w504:string, "error out"=w501:errorcluster)  [unwired: 5 in, 2 out]
            n191 = call <instrlib>:"Real 32 Converter.vi"("Data In"=w504) -> ("Data Array Out"=w503:sgl[])  [unwired: 10 in]
          }
          frame True {
          }
        }
      }
    }
    n192 = local read "Drain Source Channel"() -> (w452:T1)
    n193 = Empty Array?(array=w432) -> (empty?=w431:bool)
    n194 = case shown="False" w431 {
      tunnel: w435 -> [w469 _]
      tunnel: w432 -> [w468 _]
      frame False {
        n195 = Lossy Enqueue Element(queue=w469, element=w468) -> (overflow?=→"Overflow?":bool)  [unwired: 1 in, 3 out]
      }
      frame True {
      }
    }
    n196 = call <instrlib>:"Event Module Overrun.vi"("Channel (Channel A)"=w452, "error in"=w434, "Event Module Type (Digital I/O)"=T5."Measure", "VISA resource name"=w454) -> ("error out"=w433:errorcluster, "Overrun?"=→"Overrun?":bool, "VISA resource name out"=w439:refnum<visa-resource-name>)  [unwired: 3 in, 2 out]
    n197 = Or(x=w438, y="Stop") -> (x .or. y?=w440:bool)
  }
  n198 = Release Queue(queue=w51) -> (error out=w48:errorcluster)  [unwired: 2 in, 2 out]
  n199 = Decimate 1D Array(w40) -> (w4:sgl[], w5:sgl[])  [unwired: 1 out]
  n200 = call "Convert to Dynamic Data9"("Array"=w4) -> ("Dynamic Data Type"=w2:dynamicdata)  [unwired: 3 in]
  n201 = call "Convert to Dynamic Data8"("Array"=w5) -> ("Dynamic Data Type"=w1:dynamicdata)  [unwired: 3 in]
  n202 = call "Build XY Graph4"("Y Input"=w2, "X Input"=w1) -> ("XY Graph"=w3:cluster{"X":dbl[], "Y":dbl[]}[])  [unwired: 8 in, 1 out]
  n203 = local write "EPSC"(w3) -> ()
  n204 = case shown="False" w76 {
    tunnel: w84 -> [w521 w523]
    tunnel: w83 -> [w520 w522]
    tunnel: [w515 w523] -> w82
    tunnel: [w514 w522] -> w81
    frame False {
      w516 = u16 1 items=["Channel A", "Channel B"] ("Channel (Channel A)")
      w517 = u16 0 items=["Channel A", "Channel B"] ("Channel (Channel A)")
      # "Abort Operation"
      n205 = call <instrlib>:"Abort SMU Op.vi"("error in"=w520, "Channel (Channel A)"=w517, "VISA resource name"=w521) -> ("error out"=w518:errorcluster, "VISA resource name out"=w519:refnum<visa-resource-name>)  [unwired: 5 in, 2 out]
      n206 = call <instrlib>:"Abort SMU Op.vi"("error in"=w518, "Channel (Channel A)"=w516, "VISA resource name"=w519) -> ("error out"=w514:errorcluster, "VISA resource name out"=w515:refnum<visa-resource-name>)  [unwired: 5 in, 2 out]
    }
    frame True {
      # "Operation Completed"
    }
  }
  n207 = local read "Auto Enable Output"() -> (w36:bool)
  n208 = case shown="False" w36 {
    tunnel: w82 -> [w525 w529]
    tunnel: w81 -> [w524 w528]
    tunnel: [w524 w527] -> w78
    tunnel: [w525 w526] -> w77
    frame False {
    }
    frame True {
      w534 = FALSE ("Output (Off)")
      n209 = local read "Drain Source Channel"() -> (w531:T1)
      n210 = local read "Pulse Channel"() -> (w530:T1)
      n211 = call <instrlib>:"Source Output Enable.vi"("Output (Off)"=w534, "error in (no error)"=w528, "Channel (Channel A)"=w531, "VISA resource name"=w529) -> ("error out"=w532:errorcluster, "VISA resource name out"=w533:refnum<visa-resource-name>)  [unwired: 4 in, 2 out]
      n212 = call <instrlib>:"Source Output Enable.vi"("Output (Off)"=w534, "error in (no error)"=w532, "Channel (Channel A)"=w530, "VISA resource name"=w533) -> ("error out"=w527:errorcluster, "VISA resource name out"=w526:refnum<visa-resource-name>)  [unwired: 4 in, 2 out]
    }
  }
  n213 = case shown="True" w76 {
    tunnel: w78 -> [w535 w554]
    tunnel: w77 -> [w536 w553]
    tunnel: [w535 w542] -> w75
    tunnel: [w536 w548] -> w74
    frame False {
      # "Operation Aborted, do nothing"
    }
    frame True {
      # "Plot and save Pulsed IV (single point)"
      n214 = local read "Pulse Number"() -> (w550:u32)
      n215 = call <instrlib>:"Print Buffer.vi"("VISA resource name"=w553, "End Index (1)"=w550, "Buffer Name(s)"="pulse_iv_table.v, pulse_iv_table.i" ("Buffer Name (buf)"), "error in (no error)"=w554, "Byte Count (1024)"=u32 4096) -> ("VISA resource name out"=w548:refnum<visa-resource-name>, "Buffer Data"=w549:string, "error out"=w543:errorcluster)  [unwired: 6 in, 2 out]
      n216 = call <instrlib>:"Real 32 Converter.vi"("Data In"=w549) -> ("Data Array Out"=w547:sgl[])  [unwired: 10 in]
      n217 = Decimate 1D Array(w547) -> (w546:sgl[], w545:sgl[])
      n218 = call "Convert to Dynamic Data2"("Array"=w545) -> ("Dynamic Data Type"=w540:dynamicdata)  [unwired: 3 in]
      n219 = call "Convert to Dynamic Data"("Array"=w546) -> ("Dynamic Data Type"=w541:dynamicdata)  [unwired: 3 in]
      n220 = Merge Signals(w541, w540) -> (w537:dynamicdata)
      n221 = call "Build XY Graph"("error in (no error)"=w543, "Y Input"=w540, "X Input"=w541) -> ("error out"=w542:errorcluster, "XY Graph"=→"Pulse IV":cluster{"X":dbl[], "Y":dbl[]}[])  [unwired: 7 in]
      n222 = call "Write To Measurement File2"("Signals"=w537, "Filename"="Pulsed IV Filename") -> ("Filename Out"=→"Pulsed IV Filename Out":path)  [unwired: 15 in, 2 out]
    }
  }
  n223 = call <instrlib>:"Close.vi"("error in (no error)"=w75, "VISA resource name"=w74) -> ("error out"=w50:errorcluster)  [unwired: 9 in]
  n224 = Merge Errors(w50, w48) -> (→"error out":errorcluster)
